vi "VIH ProjFile - Core.vi"(6 "cmd (get)":enum16{"get", "create", "load", "save", "close"}(ring), 8 "error in":errorcluster, 11 "Project file":path) -> (0 "error out":errorcluster, 3 "Project":T1)   [LabVIEW 2014]
doc: "::: VI Helpeks :::\nCopyright (c) 2000-2026 Konstantin Shifershteyn. All rights reserved."
uses:
  <resource>/objmgr/DOMUserDefRef.rc
panel:
  # "VI Helpeks\nCopyright (c) 2012-2026 Konstantin Shifershteyn"
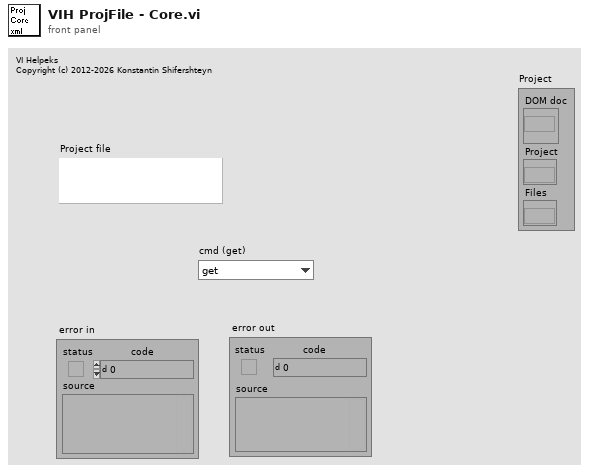
[diagram p1: front panel]
types:
  T1 = cluster{"DOM doc":refnum<k20>, "Project":refnum<k20>, "Files":refnum<k20>}
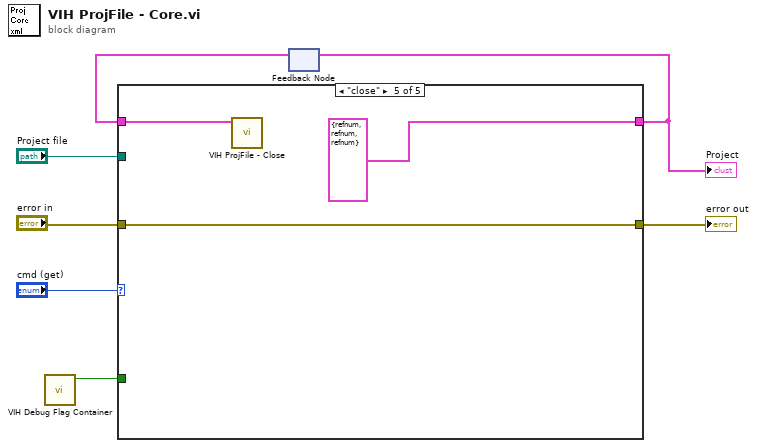
[diagram p0: block diagram]
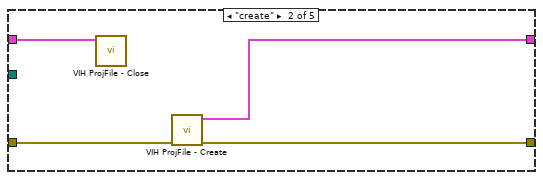
[diagram p3: hidden frame]
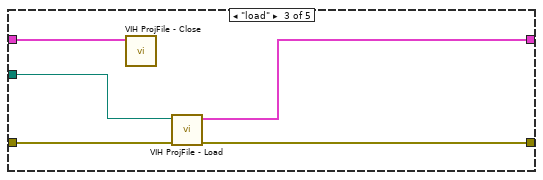
[diagram p4: hidden frame]
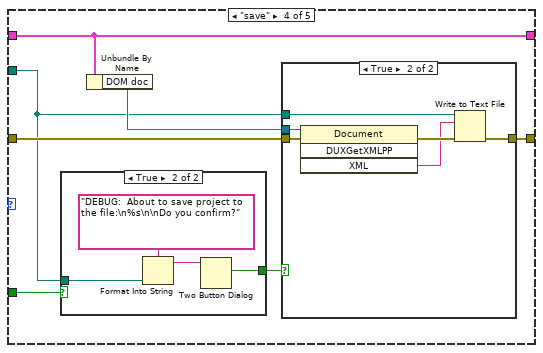
[diagram p5: hidden frame]
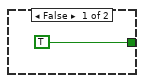
[diagram p6: hidden frame]
diagram:
  n1 = call "VIH Debug Flag Container.vi"() -> ("Debug Mode"=w1:bool)  [unwired: 11 in]
  n2 = feedback #1() -> (w3:T1)  [unwired: 1 in]
  n3 = case shown="\"close\"" "cmd (get)" {
    tunnel: "error in" -> [w8 w13 w18 w23 w38]
    tunnel: [w8 w12 w17 w22 w38] -> w5
    tunnel: [w9 w11 w16 w25 T1 {"DOM doc"=refnum, "Project"=refnum, "Files"=refnum} ("Project")] -> w4
    tunnel: w3 -> [w9 w10 w14 w25 w40]
    tunnel: "Project file" -> [_ _ w15 w19 _]
    tunnel: w1 -> [_ _ _ w20 _]
    frame "get" {
    }
    frame "create" {
      n4 = call "VIH ProjFile - Close.vi"("Project"=w10) -> ()  [unwired: 10 in, 1 out]
      n5 = call "VIH ProjFile - Create.vi"("error in"=w13) -> ("error out"=w12:errorcluster, "Project"=w11:T1)  [unwired: 9 in]
    }
    frame "load" {
      n6 = call "VIH ProjFile - Close.vi"("Project"=w14) -> ()  [unwired: 10 in, 1 out]
      n7 = call "VIH ProjFile - Load.vi"("error in"=w18, "Project File Path"=w15) -> ("error out"=w17:errorcluster, "Project"=w16:T1)  [unwired: 8 in]
    }
    frame "save" {
      n8 = case shown="True" w20 {
        tunnel: [TRUE w30] -> w21
        tunnel: w19 -> [_ w28]
        frame False {
        }
        frame True {
          n9 = Format Into String(format string="DEBUG:  About to save project to the file:\n%s\n\nDo you confirm?", w28) -> (resulting string=w27:string)  [unwired: 2 in, 1 out]
          n10 = Two Button Dialog(message=w27) -> (T button?=w30:bool)  [unwired: 2 in]
        }
      }
      n11 = Unbundle By Name(w25) -> ("DOM doc"=w24:refnum<k20>)
      n12 = case shown="True" w21 {
        tunnel: w24 -> [_ w37]
        tunnel: w23 -> [w31 w36]
        tunnel: [w31 w33] -> w22
        tunnel: w19 -> [_ w34]
        frame False {
        }
        frame True {
          n13 = invoke class="Document" method="DUXGetXMLPP"(reference=w37, error in=w36) -> (error out=w35:errorcluster, "XML"=w32:string)  [unwired: 2 in, 2 out]
          n14 = Write to Text File(file (use dialog)=w34, text=w32, error in=w35) -> (error out=w33:errorcluster)  [unwired: 1 in, 2 out]
        }
      }
    }
    frame "close" {
      n15 = call "VIH ProjFile - Close.vi"("Project"=w40) -> ()  [unwired: 10 in, 1 out]
    }
  }
  "Project" <- w4
  "error out" <- w5
  n16 = feedback-in #1(w4) -> ()
